vi "SET_UserLayers.vi"(8 "error in":errorcluster, 10 "Layers":refnum<class "Layer.lvclass">[](array[class]), 11 "Icon.lvclass in":refnum<class "Icon.lvclass">) -> (0 "error out":errorcluster, 3 "Icon.lvclass out":refnum<class "Icon.lvclass">)   [LabVIEW 2020, in "Icon.lvclass"]
doc: "Sets all User Layers."
uses:
  Icon.lvclass
  Layer/Layer.lvclass
  Icon.lvclass/Icon.ctl
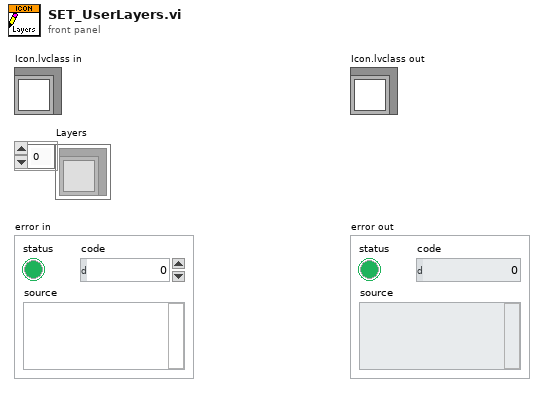
[diagram p1: front panel]
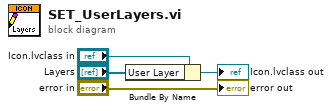
[diagram p0: block diagram]
diagram:
  n1 = Bundle By Name(cluster="Icon.lvclass in", "User Layer"="Layers") -> (→"Icon.lvclass out":refnum<class "Icon.lvclass">)
  "error out" <- "error in"
